vi "query HO Operation Band.vi"(8 "error in (no error)":errorcluster caption="에러 입력(에러 없음)", 10 "Selected CC Argements":T1, 11 "NR 입력":refnum<class "NR.lvclass">) -> (0 "error out":errorcluster caption="에러 출력", 2 "Operation Band":u32, 3 "NR 출력":refnum<class "NR.lvclass">)   [LabVIEW 2023, in "ANRITSU Call Box.lvlib" / "NR.lvclass"]
uses:
  NR.lvclass
  NR.lvclass/NR.ctl
  ANRITSU Call Box.lvlib
  Type Definition/NR Selected CC Type Arguments.ctl
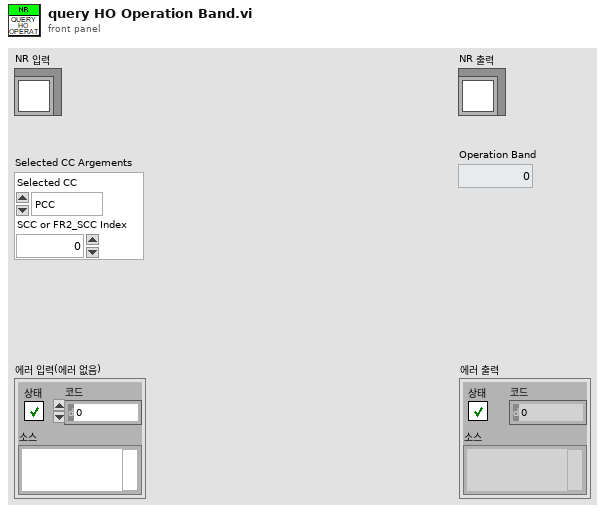
[diagram p1: front panel]
types:
  T1 = typedef "ANRITSU Call Box.lvlib/NR Selected CC Type Arguments.ctl" = cluster{"Selected CC":enum16{"PCC", "SCC", "FR2_PCC", "FR2_SCC"}, "SCC or FR2_SCC Index":u32}
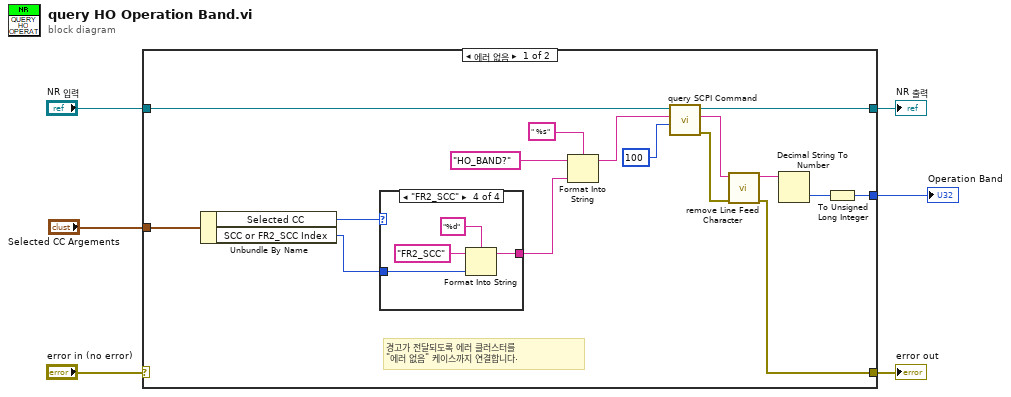
[diagram p0: block diagram]
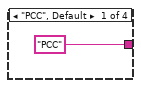
[diagram p2: hidden frame]
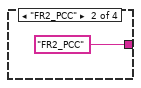
[diagram p3: hidden frame]
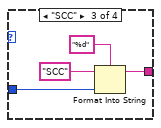
[diagram p4: hidden frame]
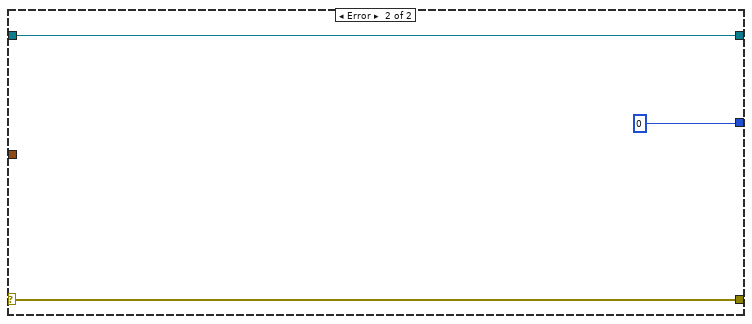
[diagram p5: hidden frame]
diagram:
  n1 = case shown="에러 없음" "error in (no error)" {
    selector: "error in (no error)" -> [_ w35]
    tunnel: [w10 w35] -> w5
    tunnel: [w11 w34] -> w3
    tunnel: "NR 입력" -> [w12 w34]
    tunnel: "Selected CC Argements" -> [w9 _]
    tunnel: [w7 u32 0] -> w1
    frame No Error {
      # "경고가 전달되도록 에러 클러스터를\n\"에러 없음\" 케이스까지 연결합니다."
      n2 = Unbundle By Name(w9) -> ("Selected CC"=w8:enum16{"PCC", "SCC", "FR2_PCC", "FR2_SCC"}, "SCC or FR2_SCC Index"=w22:u32)
      n3 = case shown="\"FR2_SCC\"" w8 {
        tunnel: ["PCC" "FR2_PCC" w26 w30] -> w20
        tunnel: w22 -> [_ _ w25 w29]
        frame "PCC", Default {
        }
        frame "FR2_PCC" {
        }
        frame "SCC" {
          n4 = Format Into String(format string="%d", initial string="SCC", w25) -> (resulting string=w26:string)  [unwired: 1 in, 1 out]
        }
        frame "FR2_SCC" {
          n5 = Format Into String(format string="%d", initial string="FR2_SCC", w29) -> (resulting string=w30:string)  [unwired: 1 in, 1 out]
        }
      }
      n6 = Format Into String(format string=" %s", initial string="HO_BAND?", w20) -> (resulting string=w18:string)  [unwired: 1 in, 1 out]
      n7 = call "query SCPI Command.vi"("Read Buffer Length"=u32 100, "SCPI Command"=w18, "NR in"=w12) -> ("error out"=w15:errorcluster, "Read Buffer String"=w16:string, "NR out"=w11:refnum<class "NR.lvclass">)  [unwired: 6 in]
      n8 = call "remove Line Feed Character.vi"("error in"=w15, "Query String"=w16) -> ("error out"=w10:errorcluster, "Line Feed Removed String"=w13:string)  [unwired: 8 in]
      n9 = Decimal String To Number(string=w13) -> (number=w14:i32)  [unwired: 2 in, 1 out]
      n10 = To Unsigned Long Integer(number=w14) -> (unsigned 32bit integer=w7:u32)
    }
    frame Error {
    }
  }
  "error out" <- w5
  "NR 출력" <- w3
  "Operation Band" <- w1
